vi "Set Slot.vi"(8 "error in":errorcluster, 10 "module":refnum<class "Module.lvclass">, 11 "slot ref in":T2 format="%.0x") -> (0 "error out":errorcluster, 3 "slot ref out":T2 format="%.0x")   [LabVIEW 2027, in "Scan Engine Scripting.lvlib"]
doc: "Writes a module configuration for a slot."
uses:
  Scan Engine Scripting.lvlib
  Modules/Mode Classes/Mode/Mode.lvclass
  Shared/SEECD Shared.lvlib
  <vilib>/regexp/Match Regular Expression.xnode
  Shared/Globals/Error Strings.vi
  Includes/Modules.lvlibp/9224/9224.lvclass
  Modules/NI 9224/NI 9224.lvclass
  Modules/NI 9228/NI 9228.lvclass
  Modules/NI 9212/NI 9212.lvclass
  Includes/Modules.lvlibp/9212/9212.lvclass
  Includes/Modules.lvlibp/9213/9213.lvclass
  Modules/NI 9213/NI 9213.lvclass
  Modules/Module/Module.lvclass
  <vilib>/NI VeriStand/Custom Device API/Custom Device Item Ref.ctl
  <vilib>/NI VeriStand/Custom Device API/Custom Device API.lvlib
  Includes/Modules.lvlibp/RSI Module/Module Models.ctl
panel:
  in  "module model":T1
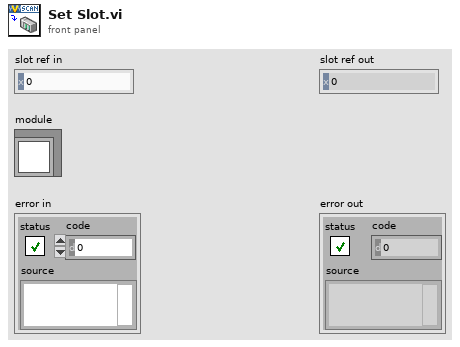
[diagram p1: front panel]
types:
  T1 = typedef "Modules.lvlibp/RSI Module.lvclass/Module Models.ctl" = enum16{"Empty", "NI 9201", "NI 9203", "NI 9205", "NI 9206", "NI 9207", "NI 9208", "NI 9209", "NI 9210", "NI 9211", "NI 9212", "NI 9213", "NI 9214", "NI 9215", "NI 9216", "NI 9217", "NI 9219", "NI 9220", "NI 9221", "NI 9222", "NI 9223", "NI 9224", "NI 9225", "NI 9226", "NI 9227", "NI 9228", "NI 9229", "NI 9233", "NI 9234", "NI 9235", "NI 9236", "NI 9237", "NI 9239", "NI 9242", "NI 9244", "NI 9253", "NI 9263", "NI 9264", "NI 9265", "NI 9266", "NI 9269", "NI 9344", "NI 9350", "NI 9375", "NI 9401", "NI 9402", "NI 9403", "NI 9411", "NI 9421", "NI 9422", "NI 9423", "NI 9425", "NI 9426", "NI 9435", "NI 9436", "NI 9437", "NI 9472", "NI 9474", "NI 9475", "NI 9476", "NI 9477", "NI 9478", "NI 9481", "NI 9482", "NI 9485"}
  T2 = typedef "Custom Device API.lvlib/Custom Device Item Ref.ctl" = u64
  T3 = typedef "Modules.lvlibp/Custom Device API.lvlib/Custom Device Item Ref.ctl" = u64
  T4 = typedef "Modules.lvlibp/RSI Module.lvclass/Slot Settings.ctl" = cluster{"Slot":u32, "EtherCAT?":bool}
  T5 = typedef "Scan Engine Scripting.lvlib/Conversion Time.ctl" = enum16{"High Speed (1k S/s)", "Medium Speed (100 S/s)", "Medium Resolution (50/60Hz Rejection - 12 S/s)", "High Resolution (50/60Hz Rejection - 2 S/s)"}
  T6 = typedef "Scan Engine Scripting.lvlib/Thermocouple Channel.lvclass/Measurement Units.ctl" = enum16{"Raw Volts", "Degrees Kelvin", "Degrees Celsius", "Degrees Fahrenheit", "Degrees Rankine"}
  T7 = typedef "Scan Engine Scripting.lvlib/Thermocouple Channel.lvclass/Thermocouple Type.ctl" = enum16{"J", "K", "T", "E", "R", "S", "N", "B"}
  T8 = typedef "Scan Engine Scripting.lvlib/NI 9212.lvclass/NI 9212 Conversion Time.ctl" = enum16{"High Speed", "Best 60 Hz Rejection", "Best 50 Hz Rejection", "High Resolution"}
  T9 = typedef "Scan Engine Scripting.lvlib/NI 9213.lvclass/NI 9213 Conversion Time.ctl" = enum16{"High Speed", "High Resolution"}
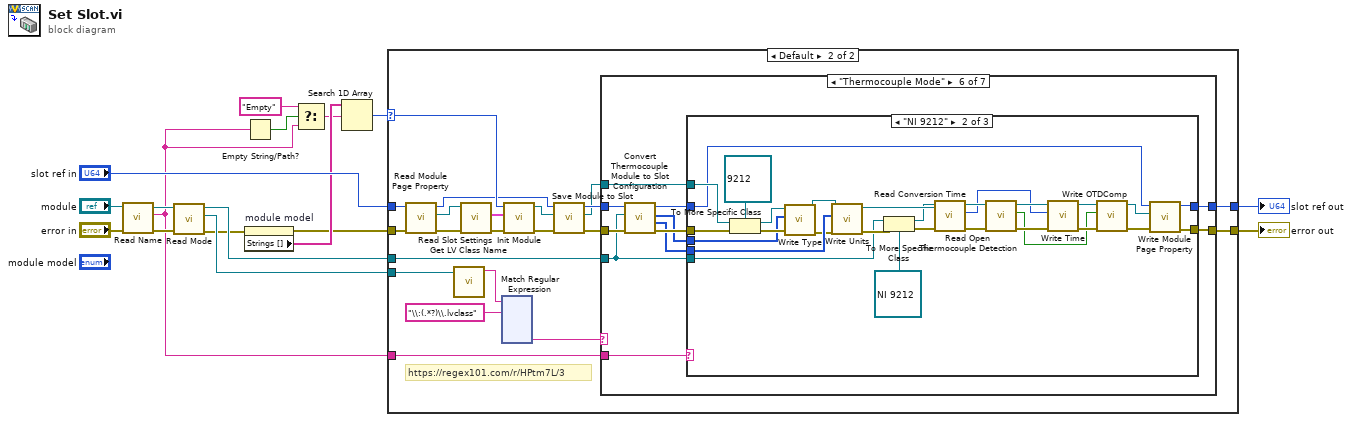
[diagram p0: block diagram]
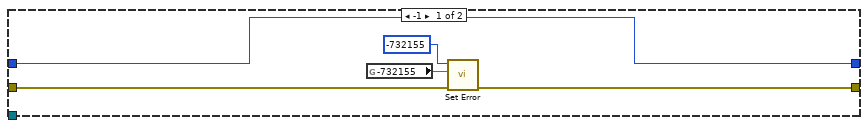
[diagram p2: hidden frame]
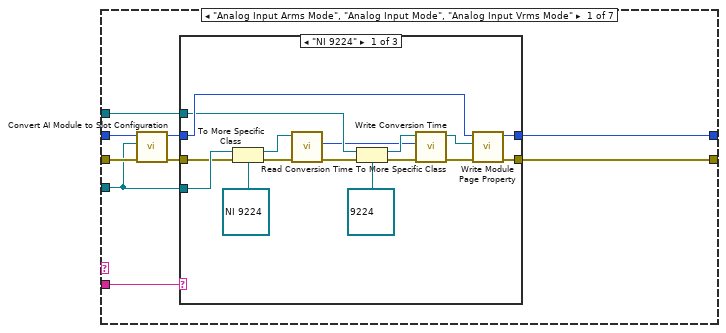
[diagram p3: hidden frame]
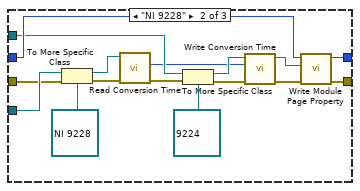
[diagram p4: hidden frame]
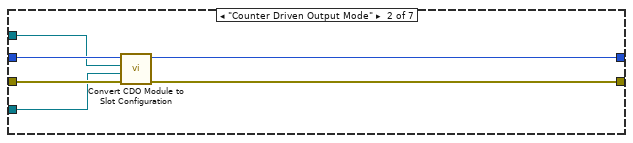
[diagram p6: hidden frame]
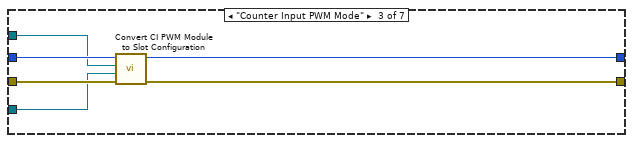
[diagram p7: hidden frame]
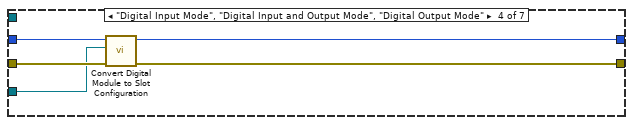
[diagram p8: hidden frame]
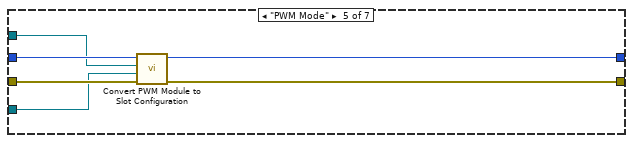
[diagram p9: hidden frame]
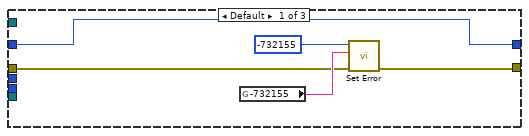
[diagram p10: hidden frame]
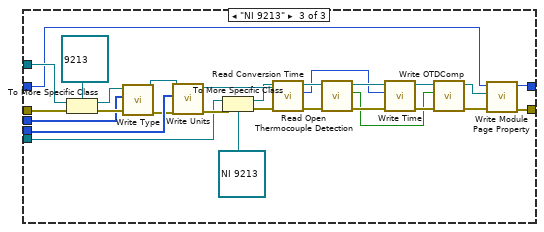
[diagram p11: hidden frame]
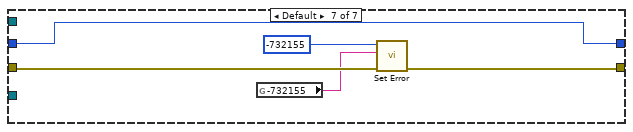
[diagram p12: hidden frame]
diagram:
  n1 = call-dynamic "Read Name.vi"("error in"="error in", "module in"="module") -> ("error out"=w6:errorcluster, "name"=w1:string, "module out"=w5:refnum<class "Module.lvclass">)  [unwired: 7 in]
  n2 = call-dynamic "Read Mode.vi"("error in"=w6, "module in"=w5) -> ("error out"=w2:errorcluster, "mode"=w4:refnum<class "Mode.lvclass">, "module out"=w3:refnum<class "Module.lvclass">)  [unwired: 7 in]
  n3 = Empty String/Path?(string/path=w1) -> (empty?=w9:bool)
  n4 = property on="module model" class="Enum (strict)"(error in=w2) -> (error out=w12:errorcluster, "Strings []"=w14:string[])  [unwired: 1 in, 1 out]
  n5 = Select(t="Empty" ("f"), s=w9, f=w1) -> (s? t:f=w8:string)
  n6 = Search 1D Array(1D array=w14, element=w8) -> (index of element=w13:i32)  [unwired: 1 in]
  n7 = case shown="Default" w13 {
    selector: w13 -> [_ w31]
    tunnel: "slot ref in" -> [w22 w39]
    tunnel: w12 -> [w18 w28]
    tunnel: [w21 w33] -> w16
    tunnel: [w22 w32] -> w15
    tunnel: w4 -> [_ w35]
    tunnel: w3 -> [_ w34]
    tunnel: w1 -> [_ w30]
    frame -1 {
      n8 = global read "Error Strings.vi" "-732155"() -> (w19:string)
      n9 = call "Set Error.vi"("error in (no error)"=w18, "Message"=w19, "Code"=-732155) -> ("error out"=w21:errorcluster)  [unwired: 8 in]
    }
    frame Default {
      # "https://regex101.com/r/HPtm7L/3"
      n10 = call "Read Module Page Property.vi"("error in (no error)"=w28, "Node Ptr In"=w39) -> ("error out"=w43:errorcluster, "RSI Module"=w42:refnum<class "RSI Module.lvclass">, "Node Ptr Out"=w26:T3)  [unwired: 7 in]
      n11 = call <vilib>:"Get LV Class Name.vi"("object"=w35) -> ("class name"=w37:string)  [unwired: 9 in, 1 out]
      n12 = call "Read Slot Settings.vi"("error in (no error)"=w43, "RSI Module in"=w42) -> ("error out"=w41:errorcluster, "Slot Settings"=w40:T4)  [unwired: 7 in, 1 out]
      n13 = xnode "Match Regular Expression"("input string"=w37, "regular expression"="\\:(.*?)\\.lvclass") -> ("submatch 1"=w36:string)  [unwired: 4 in, 5 out]
      n14 = call "Init Module.vi"("error in (no error)"=w41, "Slot Settings"=w40, "Module Model"=w31) -> ("error out"=w29:errorcluster, "RSI Module out"=w24:refnum<class "RSI Module.lvclass">)  [unwired: 7 in]
      n15 = call "Save Module to Slot.vi"("error in"=w29, "RSI module in"=w24, "slot ref in"=w26) -> ("error out"=w27:errorcluster, "RSI module out"=w23:refnum<class "RSI Module.lvclass">, "slot ref out"=w25:T3)  [unwired: 6 in]
      n16 = case shown="\"Thermocouple Mode\"" w36 {
        tunnel: w34 -> [w165 w206 w213 w218 w223 w230 _]
        tunnel: w27 -> [w170 w211 w216 w222 w228 w239 w301]
        tunnel: w23 -> [w164 w207 w212 _ w224 w236 _]
        tunnel: w25 -> [w171 w208 w217 w219 w225 w238 w303]
        tunnel: [w166 w209 w214 w221 w226 w232 w300] -> w33
        tunnel: [w168 w210 w215 w220 w227 w231 w303] -> w32
        tunnel: w30 -> [w163 _ _ _ _ w229 _]
        frame "Analog Input Arms Mode", "Analog Input Mode", "Analog Input Vrms Mode" {
          n17 = call "Convert AI Module to Slot Configuration.vi"("error in"=w170, "module in"=w165, "slot ref in"=w171) -> ("error out"=w167:errorcluster, "slot ref out"=w169:T2)  [unwired: 7 in]
          n18 = case shown="\"NI 9224\"" w163 {
            tunnel: w169 -> [w179 w195 w205]
            tunnel: [w172 w192 w205] -> w168
            tunnel: w167 -> [w186 w202 w204]
            tunnel: [w173 w193 w204] -> w166
            tunnel: w165 -> [w187 w203 _]
            tunnel: w164 -> [w178 w194 _]
            frame "NI 9224" {
              n19 = To More Specific Class(target class=refnum<class "NI 9224.lvclass"> refnum, reference=w187, error in=w186) -> (specific class reference=w177:refnum<class "NI 9224.lvclass">, error out=w176:errorcluster)
              n20 = call-dynamic "Read Conversion Time.vi"("error in"=w176, "NI 9224 in"=w177) -> ("error out"=w175:errorcluster, "conversion time"=w174:T5)  [unwired: 7 in, 1 out]
              n21 = To More Specific Class(target class=refnum<class "9224.lvclass"> refnum ("9224 in"), reference=w178, error in=w175) -> (specific class reference=w184:refnum<class "9224.lvclass">, error out=w183:errorcluster)
              n22 = call-dynamic "Write Conversion Time.vi"("error in"=w183, "Conversion Time"=w174, "9224 in"=w184) -> ("error out"=w182:errorcluster, "9224 out"=w181:refnum<class "9224.lvclass">)  [unwired: 7 in]
              n23 = call "Write Module Page Property.vi"("error in (no error)"=w182, "RSI Module"=w181, "Node Ptr In"=w179) -> ("error out"=w173:errorcluster, "Node Ptr Out"=w172:T3)  [unwired: 6 in, 1 out]
            }
            frame "NI 9228" {
              n24 = To More Specific Class(target class=refnum<class "NI 9228.lvclass"> refnum, reference=w203, error in=w202) -> (specific class reference=w191:refnum<class "NI 9228.lvclass">, error out=w190:errorcluster)
              n25 = call-dynamic "Read Conversion Time.vi"("error in"=w190, "NI 9228 in"=w191) -> ("error out"=w189:errorcluster, "conversion time"=w188:T5)  [unwired: 7 in, 1 out]
              n26 = To More Specific Class(target class=refnum<class "9224.lvclass"> refnum ("9224 in"), reference=w194, error in=w189) -> (specific class reference=w200:refnum<class "9224.lvclass">, error out=w199:errorcluster)
              n27 = call-dynamic "Write Conversion Time.vi"("error in"=w199, "Conversion Time"=w188, "9224 in"=w200) -> ("error out"=w198:errorcluster, "9224 out"=w197:refnum<class "9224.lvclass">)  [unwired: 7 in]
              n28 = call "Write Module Page Property.vi"("error in (no error)"=w198, "RSI Module"=w197, "Node Ptr In"=w195) -> ("error out"=w193:errorcluster, "Node Ptr Out"=w192:T3)  [unwired: 6 in, 1 out]
            }
            frame Default {
            }
          }
        }
        frame "Counter Driven Output Mode" {
          n29 = call "Convert CDO Module to Slot Configuration.vi"("error in"=w211, "module in"=w206, "RSI module in"=w207, "slot ref in"=w208) -> ("error out"=w209:errorcluster, "slot ref out"=w210:T2)  [unwired: 6 in]
        }
        frame "Counter Input PWM Mode" {
          n30 = call "Convert CI PWM Module to Slot Configuration.vi"("error in"=w216, "module"=w213, "RSI module"=w212, "slot ref in"=w217) -> ("error out"=w214:errorcluster, "slot ref out"=w215:T2)  [unwired: 6 in]
        }
        frame "Digital Input Mode", "Digital Input and Output Mode", "Digital Output Mode" {
          n31 = call "Convert Digital Module to Slot Configuration.vi"("error in"=w222, "module"=w218, "slot ref in"=w219) -> ("error out"=w221:errorcluster, "slot ref out"=w220:T2)  [unwired: 7 in]
        }
        frame "PWM Mode" {
          n32 = call "Convert PWM Module to Slot Configuration.vi"("error in"=w228, "module"=w223, "RSI module"=w224, "slot ref in"=w225) -> ("error out"=w226:errorcluster, "slot ref out"=w227:T2)  [unwired: 6 in]
        }
        frame "Thermocouple Mode" {
          n33 = call "Convert Thermocouple Module to Slot Configuration.vi"("error in"=w239, "module"=w230, "slot ref in"=w238) -> ("error out"=w237:errorcluster, "channel measurement units"=w233:T6[], "channel thermocouple types"=w235:T7[], "slot ref out"=w234:T2)  [unwired: 5 in]
          n34 = case shown="\"NI 9212\"" w229 {
            tunnel: w237 -> [w241 w271 w298]
            tunnel: w236 -> [_ w270 w297]
            tunnel: w235 -> [_ w266 w293]
            tunnel: w234 -> [w244 w265 w292]
            tunnel: w233 -> [_ w264 w291]
            tunnel: [w240 w261 w288] -> w232
            tunnel: [w244 w260 w287] -> w231
            tunnel: w230 -> [_ w256 w283]
            frame Default {
              n35 = global read "Error Strings.vi" "-732155"() -> (w242:string)
              n36 = call "Set Error.vi"("error in (no error)"=w241, "Message"=w242, "Code"=-732155) -> ("error out"=w240:errorcluster)  [unwired: 8 in]
            }
            frame "NI 9212" {
              n37 = To More Specific Class(target class=refnum<class "9212.lvclass"> refnum ("9213 in"), reference=w270, error in=w271) -> (specific class reference=w267:refnum<class "9212.lvclass">, error out=w269:errorcluster)
              n38 = call-dynamic "Write Type.vi"("error in (no error)"=w269, "Type"=w266, "9213 in"=w267) -> ("error out"=w263:errorcluster, "9213 out"=w262:refnum<class "9212.lvclass">)  [unwired: 7 in]
              n39 = call-dynamic "Write Units.vi"("error in (no error)"=w263, "Units"=w264, "9213 in"=w262) -> ("error out"=w257:errorcluster, "9213 out"=w259:refnum<class "9212.lvclass">)  [unwired: 7 in]
              n40 = To More Specific Class(target class=refnum<class "NI 9212.lvclass"> refnum ("NI 9212 in"), reference=w256, error in=w257) -> (specific class reference=w254:refnum<class "NI 9212.lvclass">, error out=w255:errorcluster)
              n41 = call-dynamic "Read Conversion Time.vi"("error in"=w255, "NI 9212 in"=w254) -> ("error out"=w252:errorcluster, "conversion time"=w251:T8, "NI 9212 out"=w253:refnum<class "NI 9212.lvclass">)  [unwired: 7 in]
              n42 = call-dynamic "Read Open Thermocouple Detection.vi"("error in"=w252, "NI 9212 in"=w253) -> ("error out"=w250:errorcluster, "open thermocouple detection"=w245:bool)  [unwired: 7 in, 1 out]
              n43 = call-dynamic "Write Time.vi"("error in (no error)"=w250, "Conversion Time"=w251, "9213 in"=w259) -> ("error out"=w249:errorcluster, "9213 out"=w248:refnum<class "9212.lvclass">)  [unwired: 7 in]
              n44 = call-dynamic "Write OTDComp.vi"("error in (no error)"=w249, "OTDComp"=w245, "9212 in"=w248) -> ("error out"=w246:errorcluster, "9212 out"=w247:refnum<class "9212.lvclass">)  [unwired: 7 in]
              n45 = call "Write Module Page Property.vi"("error in (no error)"=w246, "RSI Module"=w247, "Node Ptr In"=w265) -> ("error out"=w261:errorcluster, "Node Ptr Out"=w260:T3)  [unwired: 6 in, 1 out]
            }
            frame "NI 9213" {
              n46 = To More Specific Class(target class=refnum<class "9213.lvclass"> refnum ("9213 in"), reference=w297, error in=w298) -> (specific class reference=w294:refnum<class "9213.lvclass">, error out=w296:errorcluster)
              n47 = call-dynamic "Write Type.vi"("error in (no error)"=w296, "Type"=w293, "9213 in"=w294) -> ("error out"=w290:errorcluster, "9213 out"=w289:refnum<class "9213.lvclass">)  [unwired: 7 in]
              n48 = call-dynamic "Write Units.vi"("error in (no error)"=w290, "Units"=w291, "9213 in"=w289) -> ("error out"=w284:errorcluster, "9213 out"=w286:refnum<class "9213.lvclass">)  [unwired: 7 in]
              n49 = To More Specific Class(target class=refnum<class "NI 9213.lvclass"> refnum ("NI 9212 in"), reference=w283, error in=w284) -> (specific class reference=w281:refnum<class "NI 9213.lvclass">, error out=w282:errorcluster)
              n50 = call-dynamic "Read Conversion Time.vi"("error in"=w282, "NI 9213 in"=w281) -> ("error out"=w279:errorcluster, "conversion time"=w278:T9, "NI 9213 out"=w280:refnum<class "NI 9213.lvclass">)  [unwired: 7 in]
              n51 = call "Read Open Thermocouple Detection.vi"("error in"=w279, "NI 9213 in"=w280) -> ("error out"=w277:errorcluster, "open thermocouple detection"=w272:bool)  [unwired: 7 in, 1 out]
              n52 = call-dynamic "Write Time.vi"("error in (no error)"=w277, "Conversion Time"=w278, "9213 in"=w286) -> ("error out"=w276:errorcluster, "9213 out"=w275:refnum<class "9213.lvclass">)  [unwired: 7 in]
              n53 = call-dynamic "Write OTDComp.vi"("error in (no error)"=w276, "OTDComp"=w272, "9213 in"=w275) -> ("error out"=w273:errorcluster, "9213 out"=w274:refnum<class "9213.lvclass">)  [unwired: 7 in]
              n54 = call "Write Module Page Property.vi"("error in (no error)"=w273, "RSI Module"=w274, "Node Ptr In"=w292) -> ("error out"=w288:errorcluster, "Node Ptr Out"=w287:T3)  [unwired: 6 in, 1 out]
            }
          }
        }
        frame Default {
          n55 = global read "Error Strings.vi" "-732155"() -> (w299:string)
          n56 = call "Set Error.vi"("error in (no error)"=w301, "Message"=w299, "Code"=-732155) -> ("error out"=w300:errorcluster)  [unwired: 8 in]
        }
      }
    }
  }
  "error out" <- w16
  "slot ref out" <- w15
